vi "Electrical Circuit Monitoring & Protection System.vi"() -> ()   [LabVIEW 2020]
doc: "R1 + R2 + (R3 parallel R4). Resistance: kOhm; voltage: V; current: mA; power: mW. Native Turkish captions initialize when the VI runs."
panel:
  out "ErrorP":bool caption="Hata 2"
  out "WarnP":bool caption="Uyar1 2"
  out "ErrorI":bool caption="Hata 1"
  out "WarnI":bool caption="Uyar1 1"
  out "WarnV":bool caption="Uyar1"
  out "PowerLED":bool caption="Güç I_11"
  out "PowerD":dbl(knob) caption="Dirençte Harcanan Güç" scale=0.0..350.0
  out "Current":dbl(knob) caption="Direnç Ak1m1" scale=0.0..15.0
  out "Voltage":dbl(knob) caption="Direnç Gerilimi" scale=0.0..32.0
  out "Info2":string caption="Bilgi 2"
  out "Info1":string caption="Bilgi 1"
  out "Status":string caption="Durum"
  out "CircuitInfo":string caption="Devre Bilgisi"
  in  "Selection":i32 caption="Direnç Seçimi" min=0 max=4 step=1
  in  "Power":bool caption="Aç"
  out "Ptotal":dbl caption="Devrede Harcanan Güç"
  out "I3":dbl caption="I3 Ak1m1"
  out "I2":dbl caption="I2 Ak1m1"
  out "I1":dbl caption="I1 Ak1m1"
  out "Req":dbl caption="E_ Deer Direnç"
  in  "Vin":dbl caption="Giri_ Gerilimi" min=0.0 max=32.0
  in  "R4":dbl caption="4. Direnç"
  in  "R3":dbl caption="3. Direnç"
  in  "R2":dbl caption="2. Direnç"
  in  "R1":dbl caption="1. Direnç"
  # "kOhm"
  # "Kapat"
  # "kOhm"
  # "kOhm"
  # "kOhm"
  # "Volt"
  # "kOhm"
  # "Volt"
  # "mA"
  # "mW"
  # "mA"
  # "mA"
  # "mA"
  # "mW"
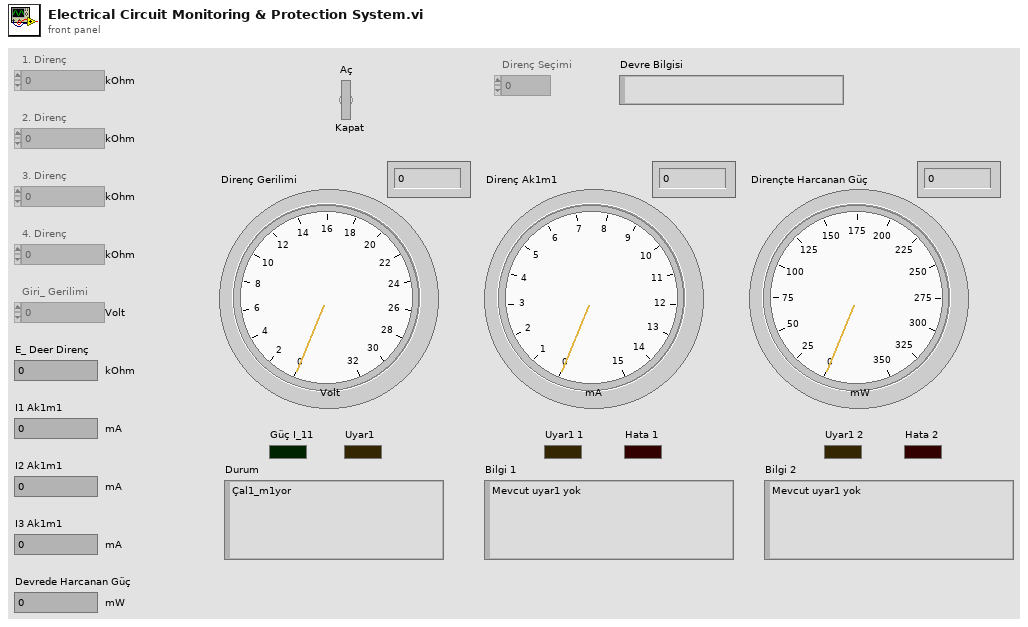
[diagram p1: front panel]
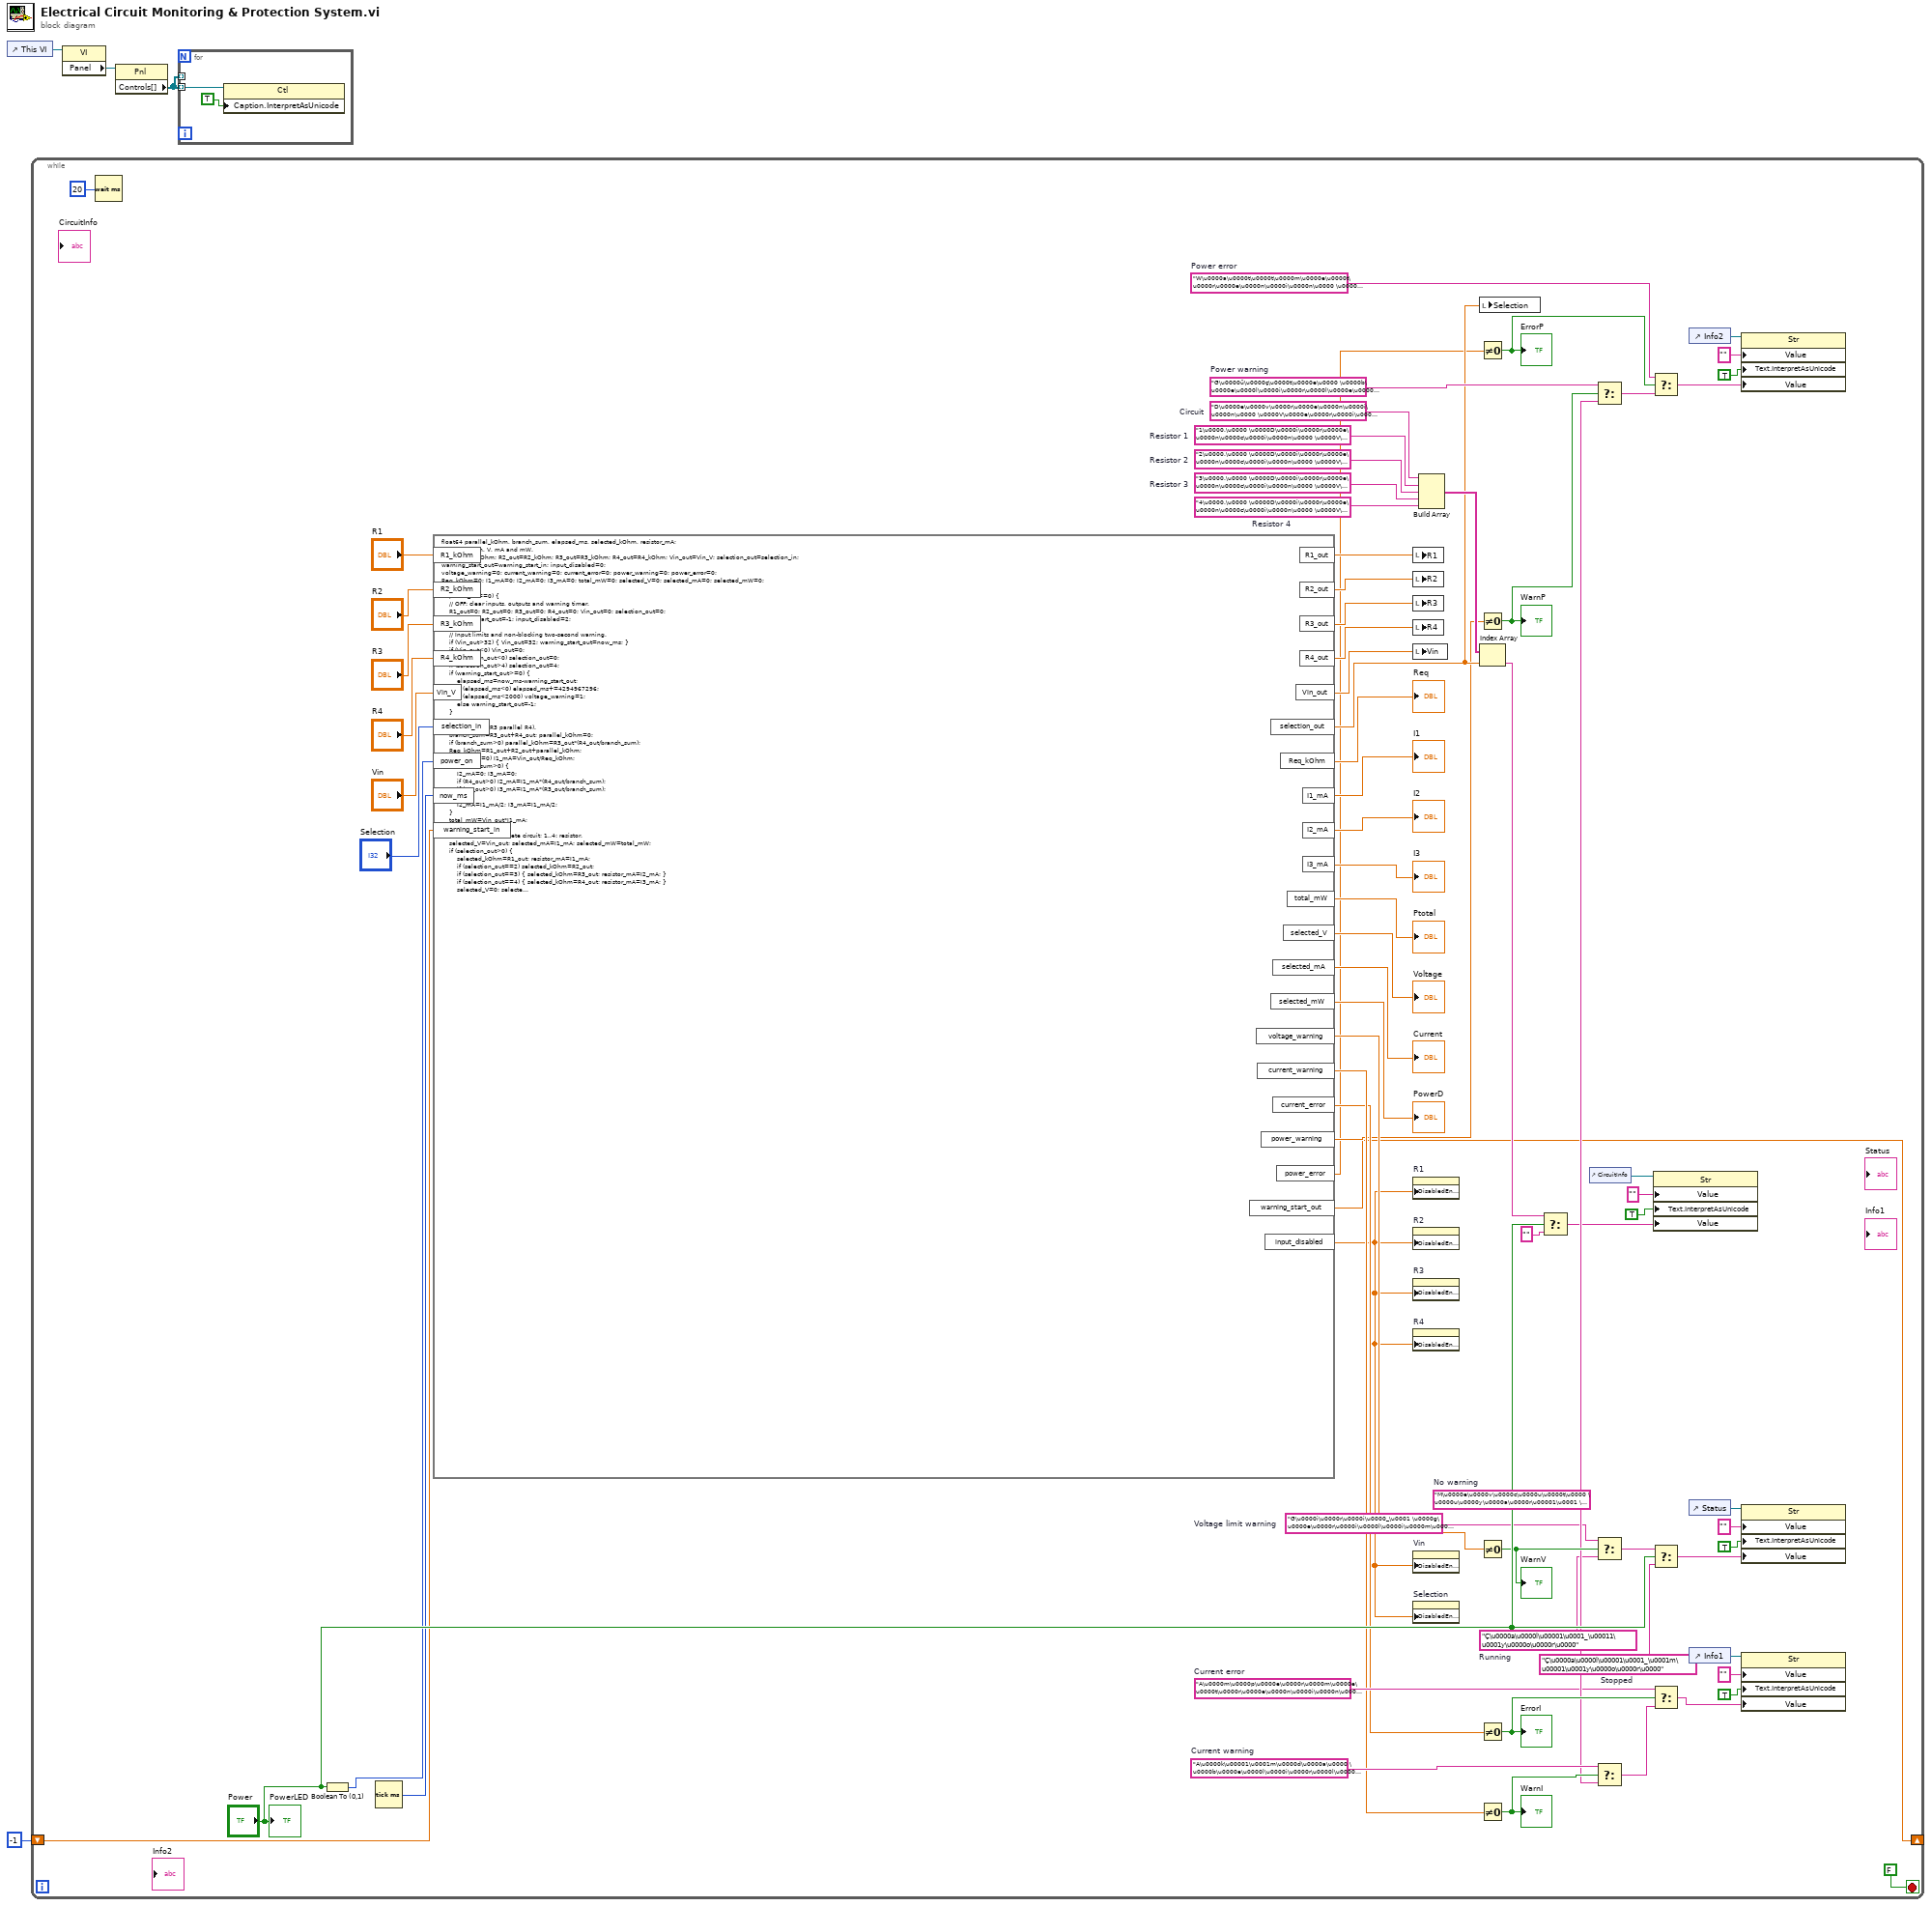
[diagram p0: block diagram]
diagram:
  n1 = control-ref of="This VI"() -> (w3:refnum<vi>)
  n2 = while {
    shift-right: [w6] -> _
    shift-left: -1 -> [w26]
    stop <- FALSE stop-if-true
    w54 = "4\u0000.\u0000 \u0000D\u0000i\u0000r\u0000e\u0000n\u0000c\u0000i\u0000n\u0000 \u0000V\u0000e\u0000r\u0000i\u0000l\u0000e\u0000r\u0000i\u0000"  # Resistor 4
    w55 = "3\u0000.\u0000 \u0000D\u0000i\u0000r\u0000e\u0000n\u0000c\u0000i\u0000n\u0000 \u0000V\u0000e\u0000r\u0000i\u0000l\u0000e\u0000r\u0000i\u0000"  # Resistor 3
    w56 = "2\u0000.\u0000 \u0000D\u0000i\u0000r\u0000e\u0000n\u0000c\u0000i\u0000n\u0000 \u0000V\u0000e\u0000r\u0000i\u0000l\u0000e\u0000r\u0000i\u0000"  # Resistor 2
    w57 = "1\u0000.\u0000 \u0000D\u0000i\u0000r\u0000e\u0000n\u0000c\u0000i\u0000n\u0000 \u0000V\u0000e\u0000r\u0000i\u0000l\u0000e\u0000r\u0000i\u0000"  # Resistor 1
    w58 = "D\u0000e\u0000v\u0000r\u0000e\u0000n\u0000i\u0000n\u0000 \u0000V\u0000e\u0000r\u0000i\u0000l\u0000e\u0000r\u0000i\u0000"  # Circuit
    w59 = "Ç\u0000a\u0000l\u00001\u0001_\u0001m\u00001\u0001y\u0000o\u0000r\u0000"  # Stopped
    w61 = "Ç\u0000a\u0000l\u00001\u0001_\u00011\u0001y\u0000o\u0000r\u0000"  # Running
    w62 = "G\u0000i\u0000r\u0000i\u0000_\u0001 \u0000g\u0000e\u0000r\u0000i\u0000l\u0000i\u0000m\u0000i\u0000 \u00003\u00002\u0000 \u0000V\u0000o\u0000l\u0000t\u0000t\u0000a\u0000n\u0000 \u0000b\u0000ü\u0000y\u0000ü\u0000k\u0000 \u0000o\u0000l\u0000a\u0000m\u0000a\u0000z\u0000"  # Voltage limit warning
    w64 = "W\u0000a\u0000t\u0000t\u0000m\u0000e\u0000t\u0000r\u0000e\u0000n\u0000i\u0000n\u0000 \u0000ö\u0000l\u0000ç\u0000e\u0000b\u0000i\u0000l\u0000e\u0000c\u0000e\u0000\u001f\u0001i\u0000 \u0000d\u0000e\u0000\u001f\u0001e\u0000r\u0000i\u0000n\u0000 \u0000d\u00001\u0001_\u00011\u0001n\u0000d\u0000a\u0000 \u0000g\u0000ü\u0000ç\u0000 \u0000h\u0000a\u0000r\u0000c\u0000a\u0000n\u00001\u0001y\u0000o\u0000r\u0000"  # Power error
    w65 = "G\u0000ü\u0000ç\u0000t\u0000e\u0000 \u0000b\u0000e\u0000l\u0000i\u0000r\u0000l\u0000e\u0000n\u0000e\u0000n\u0000 \u0000s\u00001\u0001n\u00001\u0001r\u0000 \u0000d\u0000e\u0000\u001f\u0001e\u0000r\u0000l\u0000e\u0000r\u0000i\u0000 \u0000a\u0000_\u00011\u0001l\u0000m\u0000a\u0000k\u0000 \u0000ü\u0000z\u0000e\u0000r\u0000e\u0000"  # Power warning
    w67 = "A\u0000m\u0000p\u0000e\u0000r\u0000m\u0000e\u0000t\u0000r\u0000e\u0000n\u0000i\u0000n\u0000 \u0000ö\u0000l\u0000ç\u0000e\u0000b\u0000i\u0000l\u0000e\u0000c\u0000e\u0000\u001f\u0001i\u0000 \u0000d\u0000e\u0000\u001f\u0001e\u0000r\u0000i\u0000n\u0000 \u0000d\u00001\u0001_\u00011\u0001n\u0000d\u0000a\u0000 \u0000a\u0000k\u00001\u0001m\u0000 \u0000m\u0000e\u0000v\u0000c\u0000u\u0000t\u0000"  # Current error
    w69 = "A\u0000k\u00001\u0001m\u0000d\u0000a\u0000 \u0000b\u0000e\u0000l\u0000i\u0000r\u0000l\u0000e\u0000n\u0000e\u0000n\u0000 \u0000s\u00001\u0001n\u00001\u0001r\u0000 \u0000d\u0000e\u0000\u001f\u0001e\u0000r\u0000l\u0000e\u0000r\u0000i\u0000 \u0000a\u0000_\u00011\u0001l\u0000m\u0000a\u0000k\u0000 \u0000ü\u0000z\u0000e\u0000r\u0000e\u0000"  # Current warning
    w68 = "M\u0000e\u0000v\u0000c\u0000u\u0000t\u0000 \u0000u\u0000y\u0000a\u0000r\u00001\u0001 \u0000y\u0000o\u0000k\u0000"  # No warning
    n3 = Wait (ms)(milliseconds to wait=20) -> ()  [unwired: 1 out]
    n4 = Boolean To (0,1)(Boolean="Power") -> (0, 1=w28:i16)
    n5 = Tick Count (ms)() -> (millisecond timer value=w27:u32)
    n6 = formula code="float64 parallel_kOhm, branch_sum, elapsed_ms, selected_kOhm, resistor_mA;\n// Units: kOhm, V, mA and mW.\nR1_out=R1_kOhm; R2_out=R2_kOhm; R3_out=R3_kOhm; R4_out=R4_kOhm; Vin_out=Vin_V; selection_out=selection_in;\nwarning_start_out=warning_start_in; input_disabled=0;\nvoltage_warning=0; current_warning=0; current_error=0; power_warning=0; power_error=0;\nReq_kOhm=0; I1_mA=0; I2_mA=0; I3_mA=0; total_mW=0; selected_V=0; selected_mA=0; selected_mW=0;\n\nif (power_on==0) {\n    // OFF: clear inputs, outputs and warning timer.\n    R1_out=0; R2_out=0; R3_out=0; R4_out=0; Vin_out=0; selection_out=0;\n    warning_start_out=-1; input_disabled=2;\n} else {\n    // Input limits and non-blocking two-second warning.\n    if (Vin_out>32) { Vin_out=32; warning_start_out=now_ms; }\n    if (Vin_out<0) Vin_out=0;\n    if (selection_out<0) selection_out=0;\n    if (selection_out>4) selection_out=4;\n    if (warning_start_out>=0) {\n        elapsed_ms=now_ms-warning_start_out;\n        if (elapsed_ms<0) elapsed_ms+=4294967296;\n        if (elapsed_ms<2000) voltage_warning=1;\n        else warning_start_out=-1;\n    }\n\n    // R1 + R2 + (R3 parallel R4).\n    branch_sum=R3_out+R4_out; parallel_kOhm=0;\n    if (branch_sum>0) parallel_kOhm=R3_out*(R4_out/branch_sum);\n    Req_kOhm=R1_out+R2_out+parallel_kOhm;\n    if (Vin_out!=0) I1_mA=Vin_out/Req_kOhm;\n    if (branch_sum>0) {\n        I2_mA=0; I3_mA=0;\n        if (R4_out>0) I2_mA=I1_mA*(R4_out/branch_sum);\n        if (R3_out>0) I3_mA=I1_mA*(R3_out/branch_sum);\n    } else {\n        I2_mA=I1_mA/2; I3_mA=I1_mA/2;\n    }\n    total_mW=Vin_out*I1_mA;\n\n    // Selection 0: complete circuit; 1..4: resistor.\n    selected_V=Vin_out; selected_mA=I1_mA; selected_mW=total_mW;\n    if (selection_out>0) {\n        selected_kOhm=R1_out; resistor_mA=I1_mA;\n        if (selection_out==2) selected_kOhm=R2_out;\n        if (selection_out==3) { selected_kOhm=R3_out; resistor_mA=I2_mA; }\n        if (selection_out==4) { selected_kOhm=R4_out; resistor_mA=I3_mA; }\n        selected_V=0; selected_mW=0; selected_mA=resistor_mA;\n        if (selected_kOhm!=0) { selected_V=resistor_mA*selected_kOhm; selected_mW=selected_V*resistor_mA; }\n    }\n\n    // Strict boundaries: warning >90%, error >maximum.\n    if (selected_mA>15) current_error=1;\n    else if (selected_mA>13.5) current_warning=1;\n    if (selected_mW>350) power_error=1;\n    else if (selected_mW>315) power_warning=1;\n}"("R1_kOhm"="R1", "R2_kOhm"="R2", "R3_kOhm"="R3", "R4_kOhm"="R4", "Vin_V"="Vin", "selection_in"="Selection", "power_on"=w28, "now_ms"=w27, "warning_start_in"=w26) -> ("R1_out"=w25:dbl, "R2_out"=w24:dbl, "R3_out"=w23:dbl, "R4_out"=w22:dbl, "Vin_out"=w21:dbl, "selection_out"=w20:dbl, "Req_kOhm"=→"Req":dbl, "I1_mA"=→"I1":dbl, "I2_mA"=→"I2":dbl, "I3_mA"=→"I3":dbl, "total_mW"=→"Ptotal":dbl, "selected_V"=→"Voltage":dbl, "selected_mA"=→"Current":dbl, "selected_mW"=→"PowerD":dbl, "voltage_warning"=w11:dbl, "current_warning"=w10:dbl, "current_error"=w9:dbl, "power_warning"=w8:dbl, "power_error"=w7:dbl, "warning_start_out"=w6:dbl, "input_disabled"=w5:dbl)
    n7 = local write "R1"(w25) -> ()
    n8 = local write "R2"(w24) -> ()
    n9 = local write "R3"(w23) -> ()
    n10 = local write "R4"(w22) -> ()
    n11 = local write "Vin"(w21) -> ()
    n12 = property on="R1" class="DigNum (strict)"("DisabledEnum"=w5) -> ()  [unwired: 2 in, 2 out]
    n13 = property on="R2" class="DigNum (strict)"("DisabledEnum"=w5) -> ()  [unwired: 2 in, 2 out]
    n14 = property on="R3" class="DigNum (strict)"("DisabledEnum"=w5) -> ()  [unwired: 2 in, 2 out]
    n15 = property on="R4" class="DigNum (strict)"("DisabledEnum"=w5) -> ()  [unwired: 2 in, 2 out]
    n16 = property on="Vin" class="DigNum (strict)"("DisabledEnum"=w5) -> ()  [unwired: 2 in, 2 out]
    n17 = property on="Selection" class="DigNum (strict)"("DisabledEnum"=w5) -> ()  [unwired: 2 in, 2 out]
    n18 = Build Array(w58, w57, w56, w55, w54) -> (w53:string[])
    n19 = local write "Selection"(w20) -> ()
    n20 = Not Equal To 0?(x=w7) -> (x != 0?=w70:bool)
    "ErrorP" <- w70
    n21 = Not Equal To 0?(x=w8) -> (x != 0?=w71:bool)
    "WarnP" <- w71
    n22 = Index Array(array=w53, index=w20) -> (element=w52:string)
    n23 = Not Equal To 0?(x=w11) -> (x != 0?=w74:bool)
    "WarnV" <- w74
    n24 = Not Equal To 0?(x=w9) -> (x != 0?=w72:bool)
    "ErrorI" <- w72
    n25 = Not Equal To 0?(x=w10) -> (x != 0?=w73:bool)
    "WarnI" <- w73
    n26 = Select(t=w52, s="Power", f="") -> (s? t:f=w36:string)
    n27 = control-ref of="CircuitInfo"() -> (w35:refnum<vi>)
    n28 = Select(t=w65, s=w71, f=w68) -> (s? t:f=w63:string)
    n29 = Select(t=w62, s=w74, f=w61) -> (s? t:f=w60:string)
    n30 = Select(t=w69, s=w73, f=w68) -> (s? t:f=w66:string)
    n31 = Select(t=w64, s=w70, f=w63) -> (s? t:f=w40:string)
    n32 = Select(t=w60, s="Power", f=w59) -> (s? t:f=w48:string)
    n33 = Select(t=w67, s=w72, f=w66) -> (s? t:f=w44:string)
    n34 = property class="Str"(reference=w35, "Value"="", "Text.InterpretAsUnicode"=TRUE, "Value"=w36) -> ()  [unwired: 1 in, 2 out]
    n35 = control-ref of="Info2"() -> (w39:refnum<vi>)
    n36 = control-ref of="Status"() -> (w47:refnum<vi>)
    n37 = control-ref of="Info1"() -> (w43:refnum<vi>)
    n38 = property class="Str"(reference=w39, "Value"="", "Text.InterpretAsUnicode"=TRUE, "Value"=w40) -> ()  [unwired: 1 in, 2 out]
    n39 = property class="Str"(reference=w47, "Value"="", "Text.InterpretAsUnicode"=TRUE, "Value"=w48) -> ()  [unwired: 1 in, 2 out]
    n40 = property class="Str"(reference=w43, "Value"="", "Text.InterpretAsUnicode"=TRUE, "Value"=w44) -> ()  [unwired: 1 in, 2 out]
    "PowerLED" <- "Power"
  }
  n41 = property class="VI"(reference=w3) -> ("Panel"=w2:refnum<vi>)  [unwired: 1 in, 2 out]
  n42 = property class="Pnl"(reference=w2) -> ("Controls[]"=w1:refnum<vi>[])  [unwired: 1 in, 2 out]
  n43 = for {
    tunnel: w1 -> [_] mode=indexing
    tunnel: w1 -> [w79] mode=indexing
    n44 = property class="Ctl"(reference=w79, "Caption.InterpretAsUnicode"=TRUE) -> ()  [unwired: 1 in, 2 out]
  }
